vi "update event metadata.vi"(4 "update duration":bool, 5 "type update":bool, 6 "Duration (s)":dbl, 7 "Type":T1, 8 "Labels":string[](array[string]), 9 "Description":string, 10 "Name":string, 11 "event":refnum<class "event.lvclass">) -> (0 "error out":errorcluster, 3 "updated event":refnum<class "event.lvclass">)   [LabVIEW 2020, in "nominal core steps.lvlib"]
doc: "Updates an event with additional metadata. Only populated labels and properties are used, and `type update` and `update duration` must be set to command this function to update those fields."
uses:
  nominal core steps.lvlib
  <vilib>/Nominal/Nominal IO Client/lv_src/event/event.lvclass
  <vilib>/Nominal/Nominal IO Client/lv_src/event/type.ctl
panel:
  in  "property key-value pairs":cluster{"key":string, "value":string}[](array[cluster])
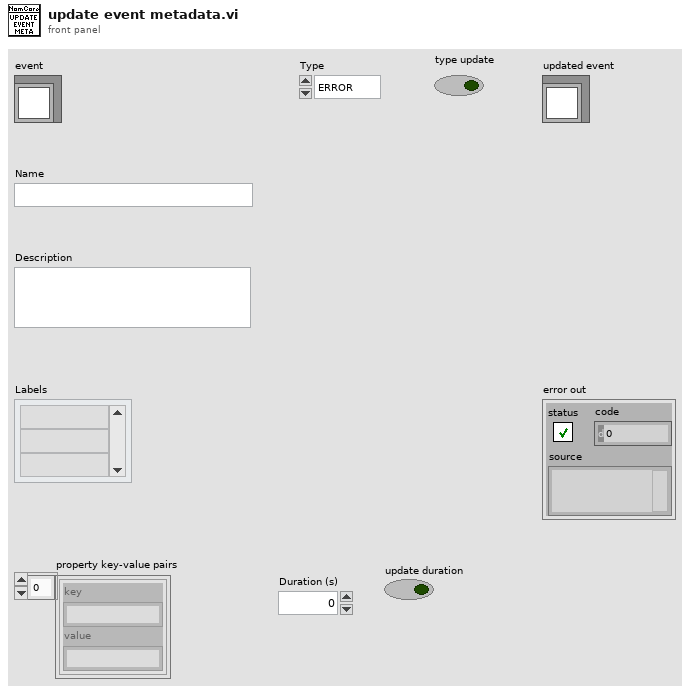
[diagram p1: front panel]
types:
  T1 = typedef "event.lvclass/type.ctl" = enum16{"ERROR", "FLAG", "INFO", "SUCCESS"}
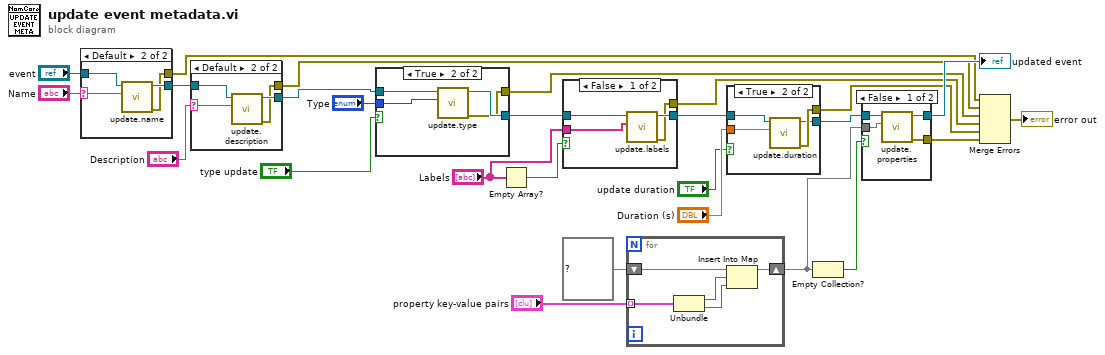
[diagram p0: block diagram]
diagram:
  n1 = case shown="Default" "Name" {
    selector: "Name" -> [_ w28]
    tunnel: "event" -> [w27 w31]
    tunnel: [w27 w30] -> w26
    tunnel: [_ w29] -> w1
    frame "" {
    }
    frame Default {
      n2 = call <vilib>:"update.name.vi"("Name"=w28, "event in"=w31) -> ("error out"=w29:errorcluster, "event out"=w30:refnum<class "event.lvclass">)  [unwired: 8 in]
    }
  }
  n3 = case shown="Default" "Description" {
    selector: "Description" -> [_ w33]
    tunnel: w26 -> [w32 w36]
    tunnel: [w32 w35] -> w25
    tunnel: [_ w34] -> w2
    frame "" {
    }
    frame Default {
      n4 = call <vilib>:"update.description.vi"("Name"=w33, "event in"=w36) -> ("error out"=w34:errorcluster, "event out"=w35:refnum<class "event.lvclass">)  [unwired: 8 in]
    }
  }
  n5 = case shown="True" "type update" {
    tunnel: w25 -> [w37 w41]
    tunnel: [w37 w40] -> w24
    tunnel: [_ w39] -> w3
    tunnel: "Type" -> [_ w38]
    frame False {
    }
    frame True {
      n6 = call <vilib>:"update.type.vi"("Type"=w38, "event in"=w41) -> ("error out"=w39:errorcluster, "event out"=w40:refnum<class "event.lvclass">)  [unwired: 8 in]
    }
  }
  n7 = Empty Array?(array="Labels") -> (empty?=w21:bool)
  n8 = case shown="False" w21 {
    tunnel: w24 -> [w45 w46]
    tunnel: [w44 w46] -> w11
    tunnel: [w43 _] -> w4
    tunnel: "Labels" -> [w42 _]
    frame False {
      n9 = call <vilib>:"update.labels.vi"("Labels"=w42, "event in"=w45) -> ("error out"=w43:errorcluster, "event out"=w44:refnum<class "event.lvclass">)  [unwired: 8 in]
    }
    frame True {
    }
  }
  n10 = for {
    tunnel: "property key-value pairs" -> [w51] mode=indexing
    shift-right: [w48] -> w15
    shift-left: map{string, string} {} ("map") -> [w49]
    n11 = Unbundle(w51) -> ("key"=w50:string, "value"=w47:string)
    n12 = Insert Into Map(map in=w49, key=w50, value=w47) -> (map out=w48:map{string, string})  [unwired: 2 out]
  }
  n13 = case shown="True" "update duration" {
    tunnel: [_ w56] -> w5
    tunnel: w11 -> [w52 w55]
    tunnel: [w52 w54] -> w10
    tunnel: "Duration (s)" -> [_ w53]
    frame False {
    }
    frame True {
      n14 = call <vilib>:"update.duration.vi"("Duration (s)"=w53, "event in"=w55) -> ("error out"=w56:errorcluster, "event out"=w54:refnum<class "event.lvclass">)  [unwired: 8 in]
    }
  }
  n15 = Empty Collection?(1:w15) -> (0:w16:bool)
  n16 = case shown="False" w16 {
    tunnel: w10 -> [w60 w61]
    tunnel: [w59 w61] -> w13
    tunnel: [w58 _] -> w19
    tunnel: w15 -> [w57 _]
    frame False {
      n17 = call <vilib>:"update.properties.vi"("properties"=w57, "event in"=w60) -> ("error out"=w58:errorcluster, "event out"=w59:refnum<class "event.lvclass">)  [unwired: 8 in]
    }
    frame True {
    }
  }
  "updated event" <- w13
  n18 = Merge Errors(w1, w2, w3, w4, w5, w19) -> (→"error out":errorcluster)
